vi "Refresh.vi"(8 "error in (no error)":errorcluster, 10 "Engine Configuration In":refnum<class "engine configuration.lvclass">, 11 "CVT editor node In":refnum<class "CVT editor node.lvclass">) -> (0 "error out":errorcluster, 2 "Engine Configuration Out":refnum<class "engine configuration.lvclass">, 3 "CVT editor node Out":refnum<class "CVT editor node.lvclass">)   [LabVIEW 2013, in "CVT editor node.lvclass"]
uses:
  CVT editor node.lvclass
  <vilib>/NI/Module Execution Interface/Engine Configuration/engine configuration.lvclass
  configuration/CVT configuration.lvclass
  <vilib>/NI/DCAF/Tag Editor Core/Configuration Editor/Classes/Module editor node/Read Module Configuration.vi
  <vilib>/NI/DCAF/Tag Editor Core/Configuration Editor/Classes/Module editor node/Write Module Configuration.vi
  <vilib>/NI/Tag Bus Module Framework/module configuration/TBM module configuration.lvclass
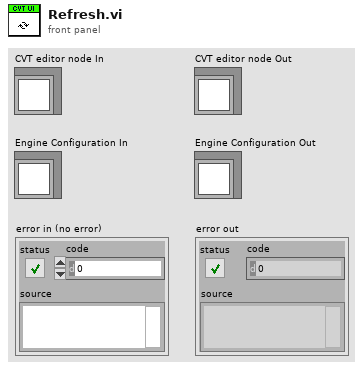
[diagram p1: front panel]
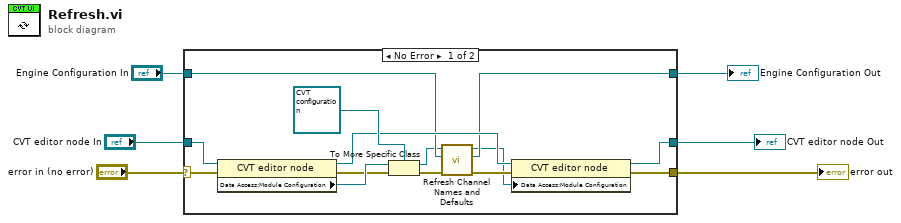
[diagram p0: block diagram]
diagram:
  n1 = case shown="No Error" "error in (no error)" {
    selector: "error in (no error)" -> [w14 w21]
    tunnel: "Engine Configuration In" -> [w9 w23]
    tunnel: "CVT editor node In" -> [w20 w22]
    tunnel: [w17 w22] -> w4
    tunnel: [w12 w21] -> w3
    tunnel: [w10 w23] -> w1
    frame No Error {
      n2 = property class="CVT editor node"(reference=w20, error in=w14) -> (reference out=w11:refnum<class "CVT editor node.lvclass">, error out=w16:errorcluster, "Data Access:Module Configuration"=w18:refnum<class "TBM module configuration.lvclass">)
      n3 = To More Specific Class(target class=refnum<class "CVT configuration.lvclass"> refnum ("CVT configuration"), reference=w18, error in=w16) -> (specific class reference=w8:refnum<class "CVT configuration.lvclass">, error out=w15:errorcluster)
      n4 = call "Refresh Channel Names and Defaults.vi"("error in (no error)"=w15, "engine configuration in"=w9, "CVT configuration in"=w8) -> ("error out"=w13:errorcluster, "engine configuration out"=w10:refnum<class "engine configuration.lvclass">, "CVT configuration out"=w7:refnum<class "CVT configuration.lvclass">)  [unwired: 6 in]
      n5 = property class="CVT editor node"(reference=w11, error in=w13, "Data Access:Module Configuration"=w7) -> (reference out=w17:refnum<class "CVT editor node.lvclass">, error out=w12:errorcluster)
    }
    frame Error {
    }
  }
  "CVT editor node Out" <- w4
  "error out" <- w3
  "Engine Configuration Out" <- w1
